vi "Get Tag.vi"(8 "error in (no error)":errorcluster, 11 "CTI_GPIO_DigitalOut in":refnum<class "CTI_GPIO_DigitalIn.lvclass">) -> (0 "error out":errorcluster, 2 "Tag":string, 3 "CTI_GPIO_DigitalOut out":refnum<class "CTI_GPIO_DigitalIn.lvclass">)   [LabVIEW 2021, in "CTI_GPIO_DigitalIn.lvclass"]
uses:
  CTI_GPIO_DigitalIn.lvclass
  CTI_GPIO_DigitalIn.lvclass/CTI_GPIO_DigitalIn.ctl
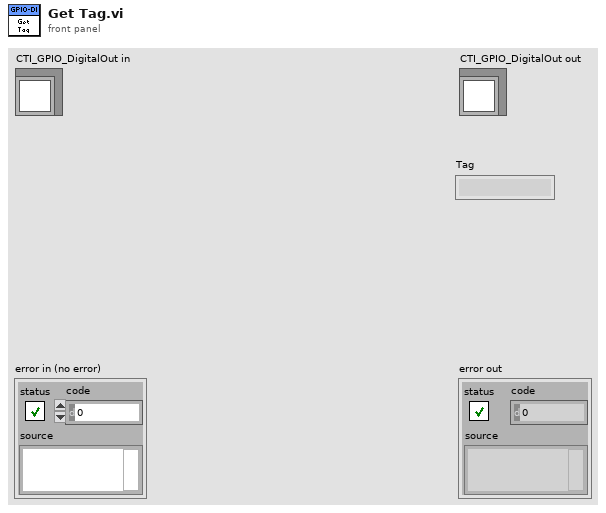
[diagram p1: front panel]
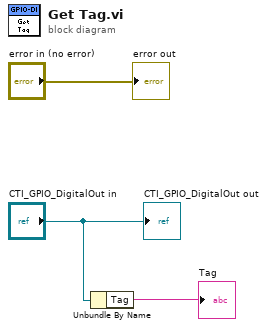
[diagram p0: block diagram]
diagram:
  n1 = Unbundle By Name("CTI_GPIO_DigitalOut in") -> ("Tag"=→"Tag":string)
  "error out" <- "error in (no error)"
  "CTI_GPIO_DigitalOut out" <- "CTI_GPIO_DigitalOut in"
